vi "ZM-PC-getTimestampString.vi"(8 "error in (no error)":errorcluster, 11 "ZM-PC-package in":refnum<class "ZM-PC-package.lvclass">) -> (0 "error out":errorcluster, 2 "timestamp_iso":string, 3 "ZM-PC-package out":refnum<class "ZM-PC-package.lvclass">)   [LabVIEW 2020, in "ZM-PC-packages.lvlib" / "ZM-PC-package.lvclass"]
doc: "Returns the package timestamp as an ISO 8601 UTC string with milliseconds (YYYY-MM-DDTHH:MM:SS.mmmZ), locale-independent: Format Date/Time String in UTC for the seconds, the fractional seconds x 1000 floored and zero-padded to three digits. Reads the field through Read timestamp."
uses:
  ZM-PC-package.lvclass
  ZM-PC-package.lvclass/ZM-PC-package.ctl
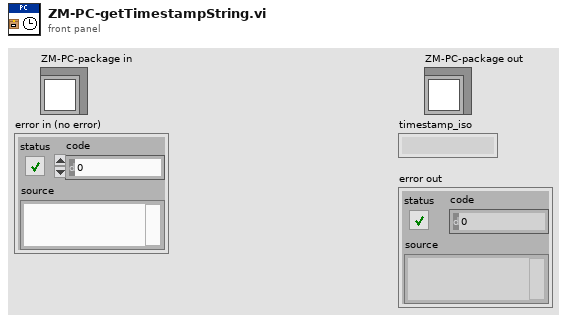
[diagram p1: front panel]
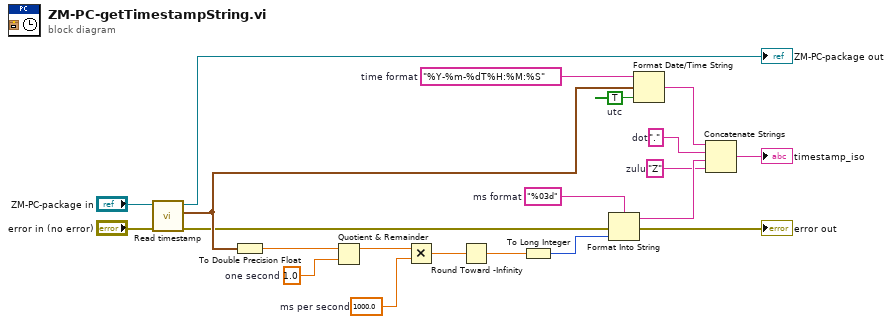
[diagram p0: block diagram]
diagram:
  w4 = "Z"  # zulu
  w6 = "."  # dot
  w10 = "%03d"  # ms format
  w13 = 1000.0  # ms per second
  w15 = 1.0  # one second
  w18 = TRUE  # utc
  w19 = "%Y-%m-%dT%H:%M:%S"  # time format
  n1 = call "Read timestamp.vi"("error in (no error)"="error in (no error)", "ZM-PC-package in"="ZM-PC-package in") -> ("error out"=w8:errorcluster, "timestamp"=w17:timestamp, "ZM-PC-package out"=→"ZM-PC-package out":refnum<class "ZM-PC-package.lvclass">)  [unwired: 7 in]
  n2 = To Double Precision Float(number=w17) -> (double precision float=w16:dbl)
  n3 = Quotient & Remainder(x=w16, y=w15) -> (x-y*floor(x/y)=w14:dbl)  [unwired: 1 out]
  n4 = Multiply(x=w14, y=w13) -> (x*y=w12:dbl)
  n5 = Round Toward -Infinity(1:w12) -> (0:w11:dbl)
  n6 = To Long Integer(number=w11) -> (32bit integer=w9:i32)
  n7 = Format Into String(format string=w10, error in=w8, w9) -> (resulting string=w5:string, error out=→"error out":errorcluster)  [unwired: 1 in]
  n8 = Format Date/Time String(time format string (%c)=w19, seconds (now)=w17, UTC format=w18) -> (date/time string=w7:string)
  n9 = Concatenate Strings(w7, w6, w5, w4) -> (→"timestamp_iso":string)
